vi "RFH-read-R140.vi"(7 "file path (dialog if empty)":path, 8 "error in (no error)":errorcluster) -> (0 "error out":errorcluster, 1 "R140 data":T2, 2 "Common Format":T1)   [LabVIEW 2020, in "RFH-Reflection_File_Handler.lvlib"]
doc: "Reads an R140 Excel file (dialog if the path is empty) and returns its data and the same data as a Common Format cluster."
uses:
  RFH-Reflection_File_Handler.lvlib
  RFH-R140_data_format.ctl
  RFH-common_data_format.ctl
  <vilib>/addons/_office/excel.llb/Excel Get Data ([dbl]).vi
  <vilib>/Utility/NIReport.llb/NI_report.lvclass
  <vilib>/Utility/NIReport.llb/Excel/NI_Excel.lvclass
  <vilib>/addons/_office/NI_ReportGenerationToolkit.lvlib
panel:
  out "Frequency":dbl[](graph)
  out "Sheet 1 Data":dbl[][](array[numeric]) format="%.2f"
  out "Output":dbl[][](array[numeric])
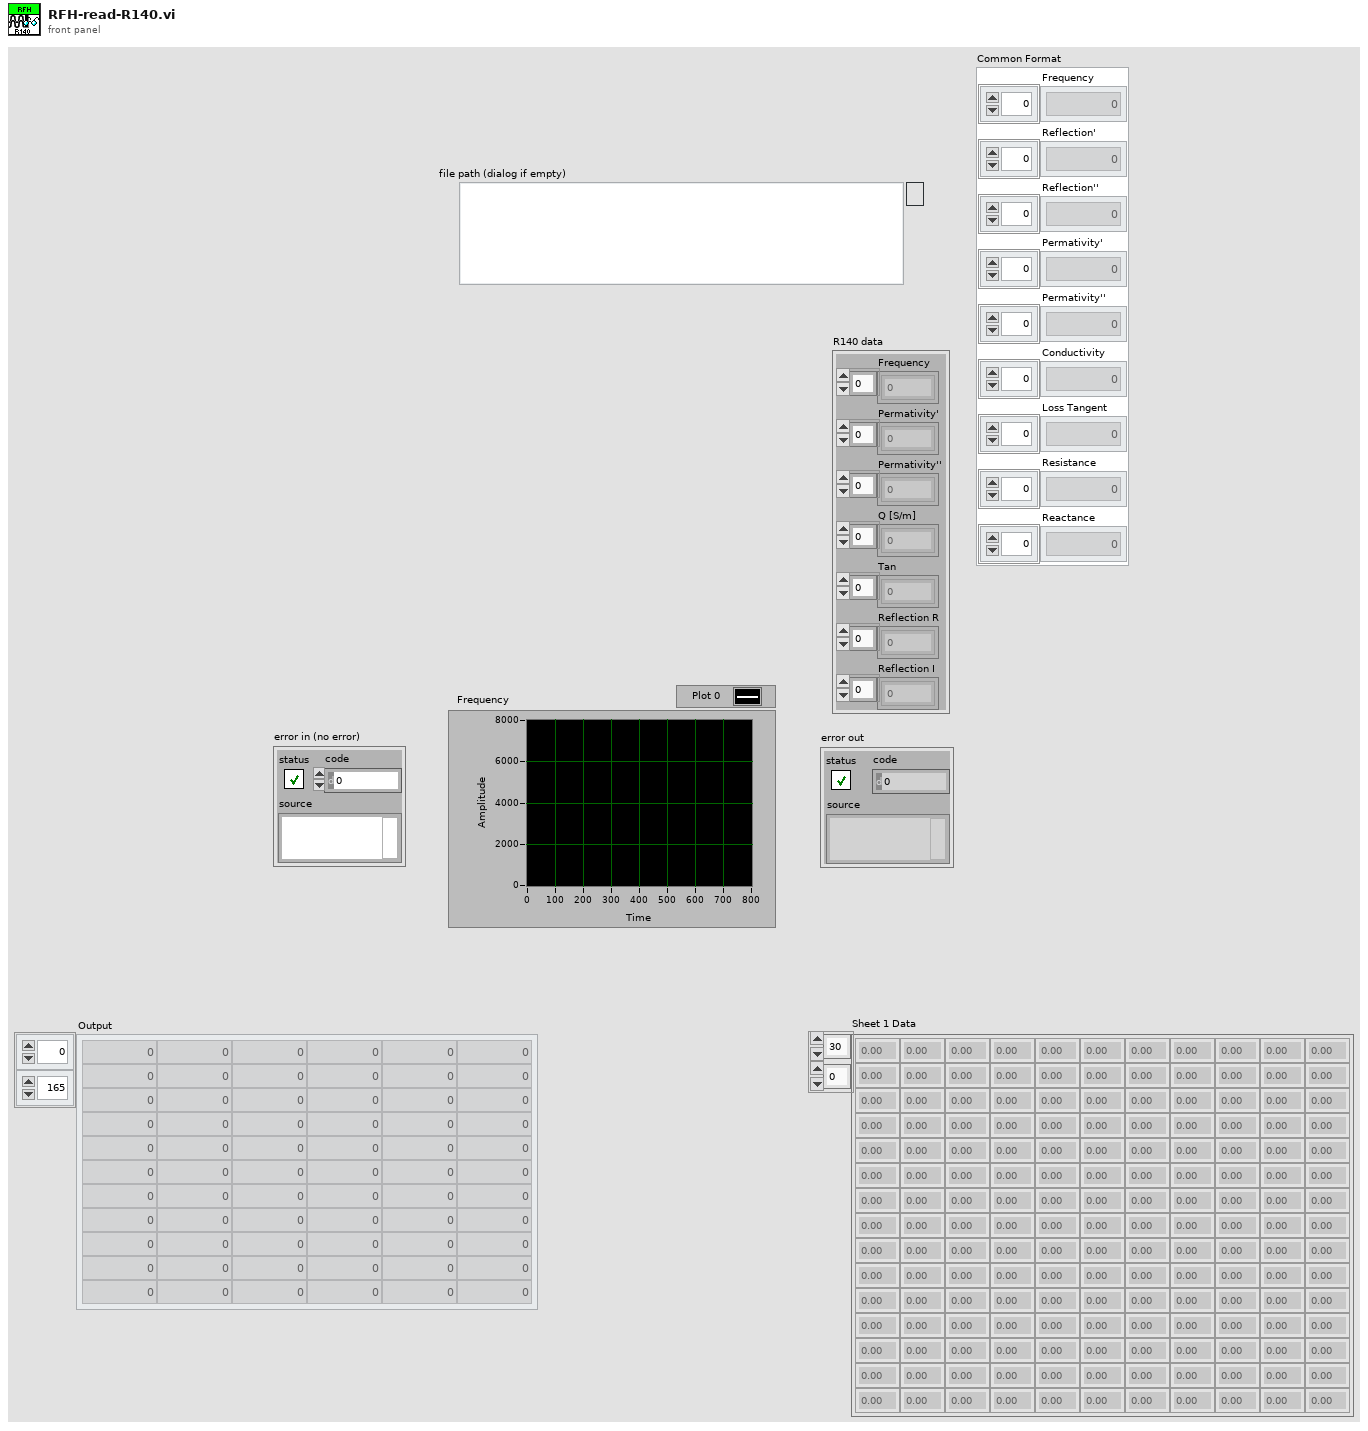
[diagram p1: front panel]
types:
  T1 = typedef "RFH-Reflection_File_Handler.lvlib/RFH-common_data_format.ctl" = cluster{"Frequency":dbl[], "Reflection'":dbl[], "Reflection''":dbl[], "Permativity'":dbl[], "Permativity''":dbl[], "Conductivity":dbl[], "Loss Tangent":dbl[], "Resistance":dbl[], "Reactance":dbl[]}
  T2 = typedef "RFH-Reflection_File_Handler.lvlib/RFH-R140_data_format.ctl" = cluster{"Frequency":dbl[], "Permativity'":dbl[], "Permativity''":dbl[], "Q [S/m]":dbl[], "Tan":dbl[], "Reflection R":dbl[], "Reflection I":dbl[]}
  T3 = enum16{"Standard Report", "HTML", "Word", "Excel"}
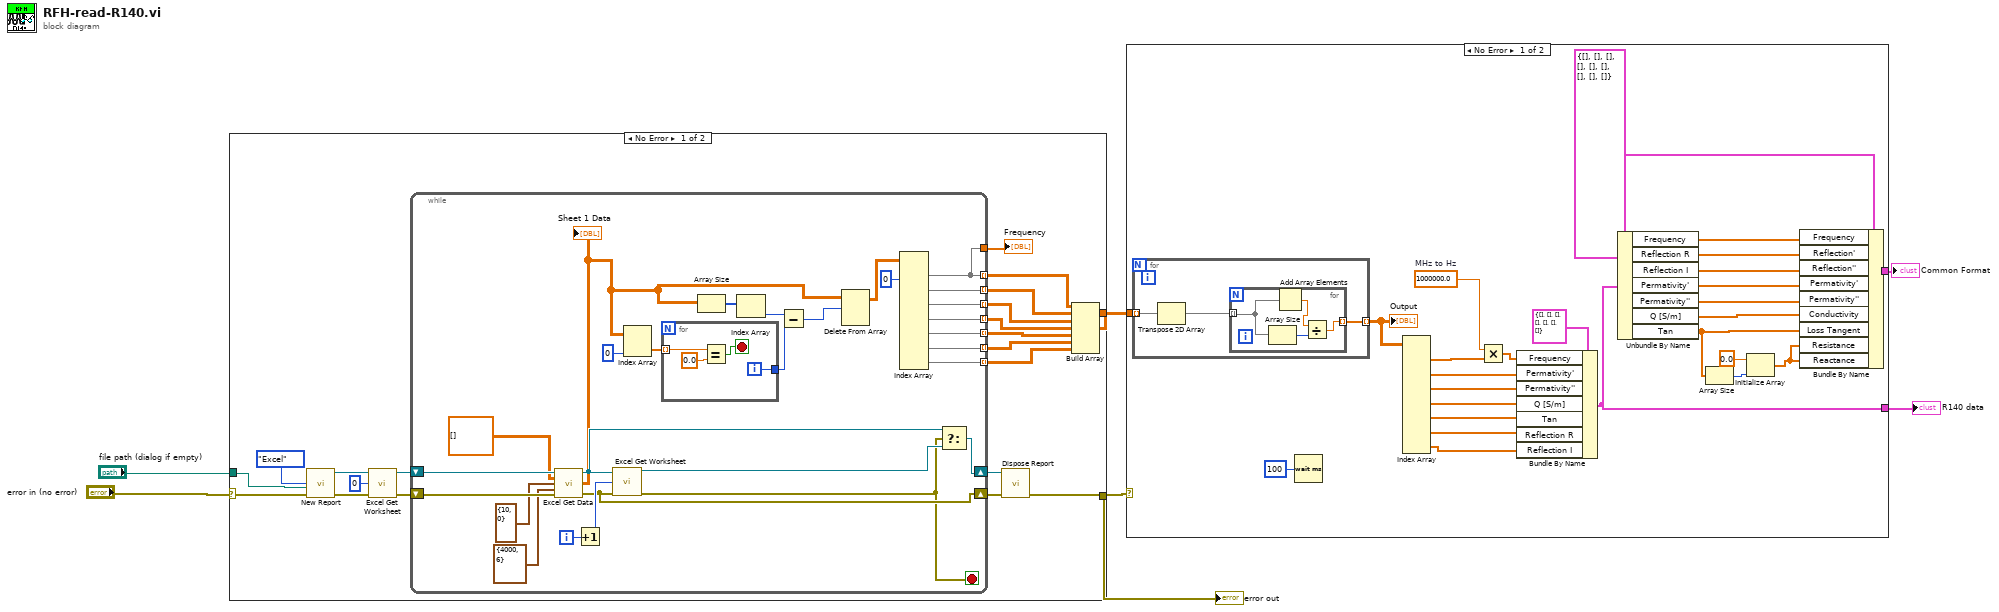
[diagram p0: block diagram]
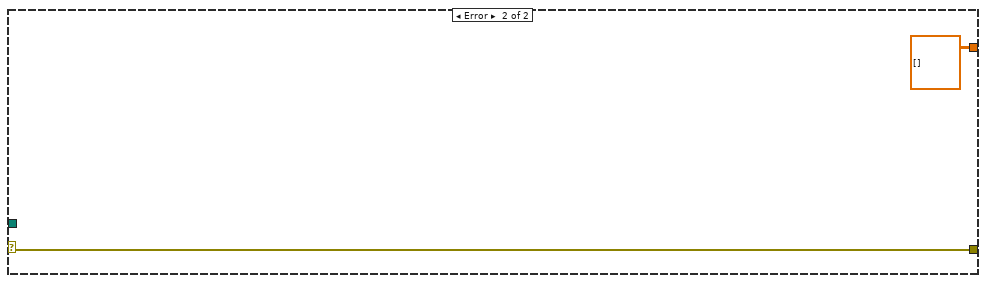
[diagram p2: hidden frame]
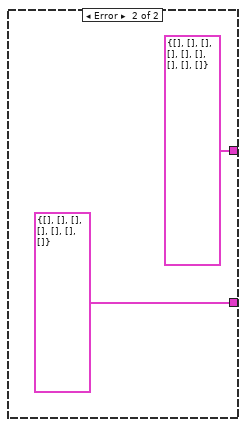
[diagram p3: hidden frame]
diagram:
  n1 = case shown="No Error" "error in (no error)" {
    selector: "error in (no error)" -> [w14 w60]
    tunnel: "file path (dialog if empty)" -> [w23 _]
    tunnel: [w20 dbl[][][] []] -> w5
    tunnel: [w7 w60] -> w1
    frame No Error {
      n2 = call <vilib>:"New Report.vi"("report type"=T3."Excel", "template (empty)"=w23, "error in (no error)"=w14) -> ("report out"=w13:refnum<class "NI_report.lvclass">, "error out"=w12:errorcluster)  [unwired: 3 in, 8 out]
      n3 = call <vilib>:"Excel Get Worksheet.vi"("report in"=w13, "worksheet index (0)"=0, "error in (no error)"=w12) -> ("report out"=w10:refnum<class "NI_report.lvclass">, "error out"=w9:errorcluster)  [unwired: 11 out]
      n4 = while {
        shift-right: [w37] -> w25
        shift-left: w10 -> [w54]
        shift-right: [w40] -> w24
        shift-left: w9 -> [w52]
        tunnel: [w35] -> w22 mode=indexing
        tunnel: [w48] -> w21 mode=indexing
        tunnel: [w47] -> w19 mode=indexing
        tunnel: [w46] -> w18 mode=indexing
        tunnel: [w45] -> w17 mode=indexing
        tunnel: [w44] -> w16 mode=indexing
        tunnel: [w43] -> w15 mode=indexing
        tunnel: [w35] -> w8
        i -> [w42]
        stop <- w36 stop-if-true
        n5 = call-poly <vilib>:"Excel Get Data.vi"("report in"=w54, "data type"=dbl[][] [], "start (-1, -1)"=cluster{"row":i32, "column":i32} {"row"=10, "column"=0}, "end (-1, -1)"=cluster{"row":i32, "column":i32} {"row"=4000, "column"=6}, "error in (no error)"=w52) -> ("report out"=w39:refnum<class "NI_report.lvclass">, "data"=w28:dbl[][], "error out"=w40:errorcluster)  [unwired: 8 out]
        "Sheet 1 Data" <- w28
        n6 = Increment(x=w42) -> (x+1=w41:i32)
        n7 = call <vilib>:"Excel Get Worksheet.vi"("report in"=w39, "worksheet index (0)"=w41, "error in (no error)"=w40) -> ("report out"=w38:refnum<class "NI_report.lvclass">, "error out"=w36:errorcluster)  [unwired: 11 out]
        n8 = Index Array(array=w28, index (col)=0 ("disabled index (col)")) -> (element=w34:dbl[])  [unwired: 1 in]
        n9 = for {
          tunnel: w34 -> [w58] mode=indexing
          tunnel: [w55] -> w30
          i -> [w55]
          stop <- w56 stop-if-true
          n10 = Equal?(x=w58, y=0.0) -> (x = y?=w56:bool)
        }
        n11 = Array Size(array=w28) -> (size(s)=w32:i32[])
        n12 = Index Array(array=w32) -> (element=w31:i32)  [unwired: 1 in]
        n13 = Subtract(x=w31, y=w30) -> (x-y=w29:i32)
        n14 = Delete From Array(array=w28, length=w29) -> (array with subset deleted=w27:dbl[][])  [unwired: 2 in, 1 out]
        n15 = Index Array(array=w27, index (col) #1=0 ("disabled index (col)")) -> (element #1=w35:dbl[], element #2=w48:dbl[], element #3=w47:dbl[], element #4=w46:dbl[], element #5=w45:dbl[], element #6=w44:dbl[], element #7=w43:dbl[])  [unwired: 13 in]
        n16 = Select(t=w39, s=w36, f=w38) -> (s? t:f=w37:refnum<class "NI_report.lvclass">)
      }
      "Frequency" <- w8
      n17 = call-dynamic "Dispose Report.vi"("report in"=w25, "error in (no error)"=w24) -> ("error out"=w7:errorcluster)  [unwired: 3 in, 10 out]
      n18 = Build Array(w22, w21, w19, w18, w17, w16, w15) -> (w20:dbl[][][])
    }
    frame Error {
    }
  }
  "error out" <- w1
  n19 = case shown="No Error" w1 {
    tunnel: w5 -> [w86 _]
    tunnel: [w74 T2 {"Frequency"=[], "Permativity'"=[], "Permativity''"=[], "Q [S/m]"=[], "Tan"=[], "Reflection R"=[], "Reflection I"=[]} ("output cluster")] -> w3
    tunnel: [w67 T1 {"Frequency"=[], "Reflection'"=[], "Reflection''"=[], "Permativity'"=[], "Permativity''"=[], "Conductivity"=[], "Loss Tangent"=[], "Resistance"=[], "Reactance"=[]} ("Common Format")] -> w2
    frame No Error {
      w75 = 1000000.0  # MHz to Hz
      n20 = for {
        tunnel: w86 -> [w87] mode=indexing
        tunnel: [w88] -> w85 mode=indexing
        n21 = Transpose 2D Array(2D array=w87) -> (transposed array=w89:dbl[][])
        n22 = for {
          tunnel: w89 -> [w93] mode=indexing
          tunnel: [w92] -> w88 mode=indexing
          n23 = Array Size(array=w93) -> (size(s)=w90:i32)
          n24 = Add Array Elements(numeric array=w93) -> (sum=w91:dbl)
          n25 = Divide(x=w91, y=w90) -> (x/y=w92:dbl)
        }
      }
      "Output" <- w85
      n26 = Wait (ms)(milliseconds to wait=u32 100) -> ()  [unwired: 1 out]
      n27 = Index Array(array=w85) -> (element #1=w84:dbl[], element #2=w83:dbl[], element #3=w82:dbl[], element #4=w81:dbl[], element #5=w80:dbl[], element #6=w79:dbl[], element #7=w78:dbl[])  [unwired: 14 in]
      n28 = Multiply(x=w75, y=w84) -> (x*y=w76:dbl[])
      n29 = Bundle By Name(cluster=T2 {"Frequency"=[], "Permativity'"=[], "Permativity''"=[], "Q [S/m]"=[], "Tan"=[], "Reflection R"=[], "Reflection I"=[]} ("output cluster"), "Frequency"=w76, "Permativity'"=w83, "Permativity''"=w82, "Q [S/m]"=w81, "Tan"=w80, "Reflection R"=w79, "Reflection I"=w78) -> (w74:T2)
      n30 = Unbundle By Name(w74) -> ("Frequency"=w72:dbl[], "Reflection R"=w71:dbl[], "Reflection I"=w70:dbl[], "Permativity'"=w69:dbl[], "Permativity''"=w68:dbl[], "Q [S/m]"=w66:dbl[], "Tan"=w63:dbl[])
      n31 = Array Size(array=w63) -> (size(s)=w65:i32)
      n32 = Initialize Array(0.0 ("element"), w65) -> (w62:dbl[])
      n33 = Bundle By Name(cluster=T1 {"Frequency"=[], "Reflection'"=[], "Reflection''"=[], "Permativity'"=[], "Permativity''"=[], "Conductivity"=[], "Loss Tangent"=[], "Resistance"=[], "Reactance"=[]} ("Common Format"), "Frequency"=w72, "Reflection'"=w71, "Reflection''"=w70, "Permativity'"=w69, "Permativity''"=w68, "Conductivity"=w66, "Loss Tangent"=w63, "Resistance"=w62, "Reactance"=w62) -> (w67:T1)
    }
    frame Error {
    }
  }
  "R140 data" <- w3
  "Common Format" <- w2
